vi "RemoteVI List Popups.vi"(0 "panel hWnd":u64) -> (4 "all popups":T1(array[cluster]), 6 "overlay popups":T1(array[cluster]), 8 "modal popups":T1(array[cluster]))   [LabVIEW 2020, in "RemoteVI.lvlib"]
doc: "Lists the LabVIEW popups open now (RemoteVI Find Popups.vi, Win32 only - no VI Server call, so it works while a popup blocks LabVIEW's UI thread) and splits them for the server loop: all popups (everything Find Popups returns), overlay popups (all but SysShadow, a menu's drop shadow, and LVTipStrip - what the OVERLAY shows; the browser shows tip strips itself from the tips message, docs\\protocol.md 3.3) and modal popups (the same list; a tip strip is not modal, so it does not switch input into popup mode). Order is kept, bottom-most first."
uses:
  RemoteVI.lvlib
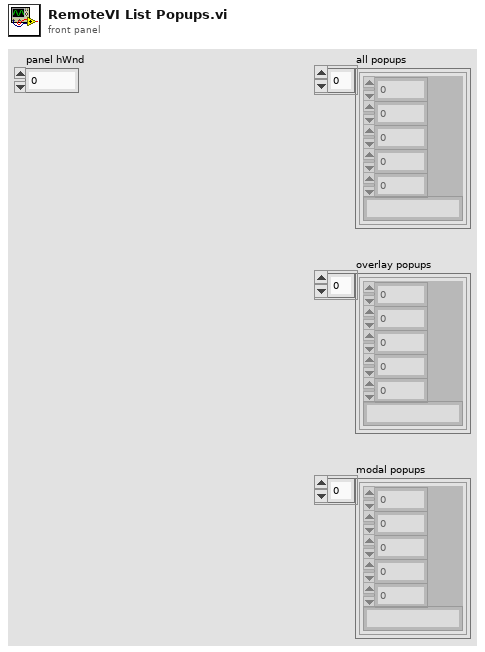
[diagram p1: front panel]
types:
  T1 = cluster{"hwnd":u64, "x":i32, "y":i32, "w":i32, "h":i32, "class":string}[]
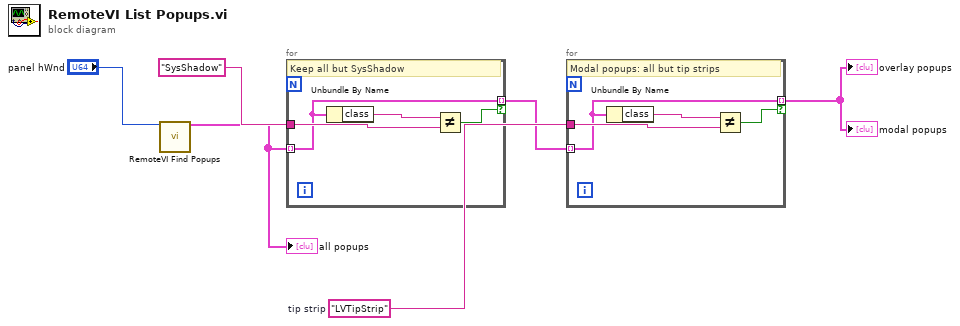
[diagram p0: block diagram]
diagram:
  w5 = "LVTipStrip"  # tip strip
  n1 = call "RemoteVI Find Popups.vi"("panel hWnd"="panel hWnd") -> ("popups"=w2:T1)  [unwired: 13 in, 1 out]
  "all popups" <- w2
  n2 = for {
    tunnel: "SysShadow" -> [w8]
    tunnel: w2 -> [w7] mode=indexing
    tunnel: [w7] -> w4 mode=indexing if=w10
    # "Keep all but SysShadow"
    n3 = Unbundle By Name(w7) -> ("class"=w9:string)
    n4 = Not Equal?(x=w9, y=w8) -> (x != y?=w10:bool)
  }
  n5 = for {
    tunnel: w5 -> [w12]
    tunnel: w4 -> [w11] mode=indexing
    tunnel: [w11] -> w6 mode=indexing if=w14
    # "Modal popups: all but tip strips"
    n6 = Unbundle By Name(w11) -> ("class"=w13:string)
    n7 = Not Equal?(x=w13, y=w12) -> (x != y?=w14:bool)
  }
  "overlay popups" <- w6
  "modal popups" <- w6
